vi "Scale Analog Input.vi"(10 "y":dbl, 11 "raw samples":dbl[](array[numeric])) -> (3 "Numeric":dbl)   [LabVIEW 2021]
uses:
  <vilib>/Analysis/baseanly.llb/Mean (DBL).vi
  <vilib>/Analysis/NI_AALBase.lvlib
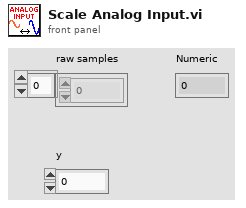
[diagram p1: front panel]
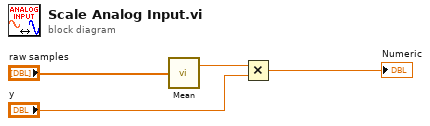
[diagram p0: block diagram]
diagram:
  n1 = call-poly <vilib>:"Mean.vi"("X"="raw samples") -> ("mean"=w2:dbl)  [unwired: 1 out]
  n2 = Multiply(x=w2, y="y") -> (x*y=→"Numeric":dbl)
